vi "RenameVI.vi"(0 "ObjectIn":refnum<class "ClassWriterNative.lvclass">, 1 "VIItemRefIn":refnum<vi>, 2 "RenameOption":T1, 5 "error in (no error)":errorcluster) -> (14 "ObjectOut":refnum<class "ClassWriterNative.lvclass">, 19 "error out":errorcluster)   [LabVIEW 2020, in "ClassWriterNative.lvclass"]
uses:
  ClassWriterNative.lvclass
  Provider_BaseClassInterface/ClassWriter_class/RenameViOption.ctl
  <vilib>/picture/picture.llb/imagedata.ctl
  Provider_BaseClassInterface/ClassWriter_class/ClassWriter.lvclass
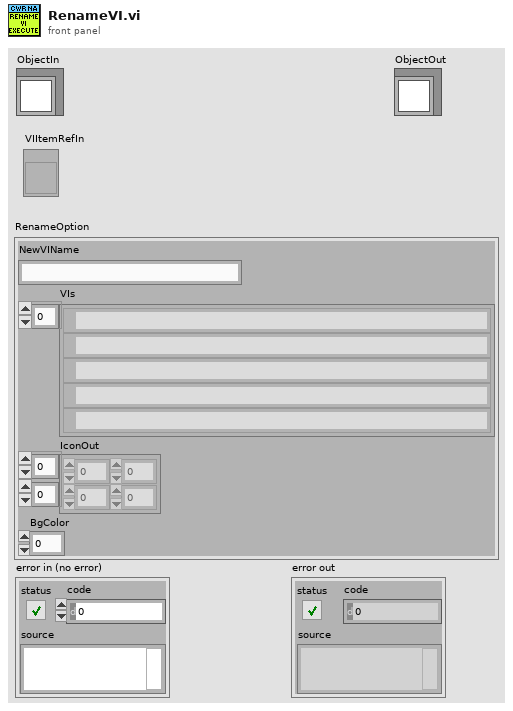
[diagram p1: front panel]
types:
  T1 = typedef "ClassWriter.lvclass/RenameViOption.ctl" = cluster{"NewVIName":string, "VIs":path[], "IconOut":u8[][], "BgColor":u8}
  T2 = cluster{"Counter":i32, "Text":string, "Cancelled":bool, "App Ref":refnum<vi>}
  T3 = typedef "imagedata.ctl" = cluster{"image type":i32, "image depth":i32, "image":u8[], "mask":u8[], "colors":u32[], "Rectangle":cluster{"left":i16, "top":i16, "right":i16, "bottom":i16}}
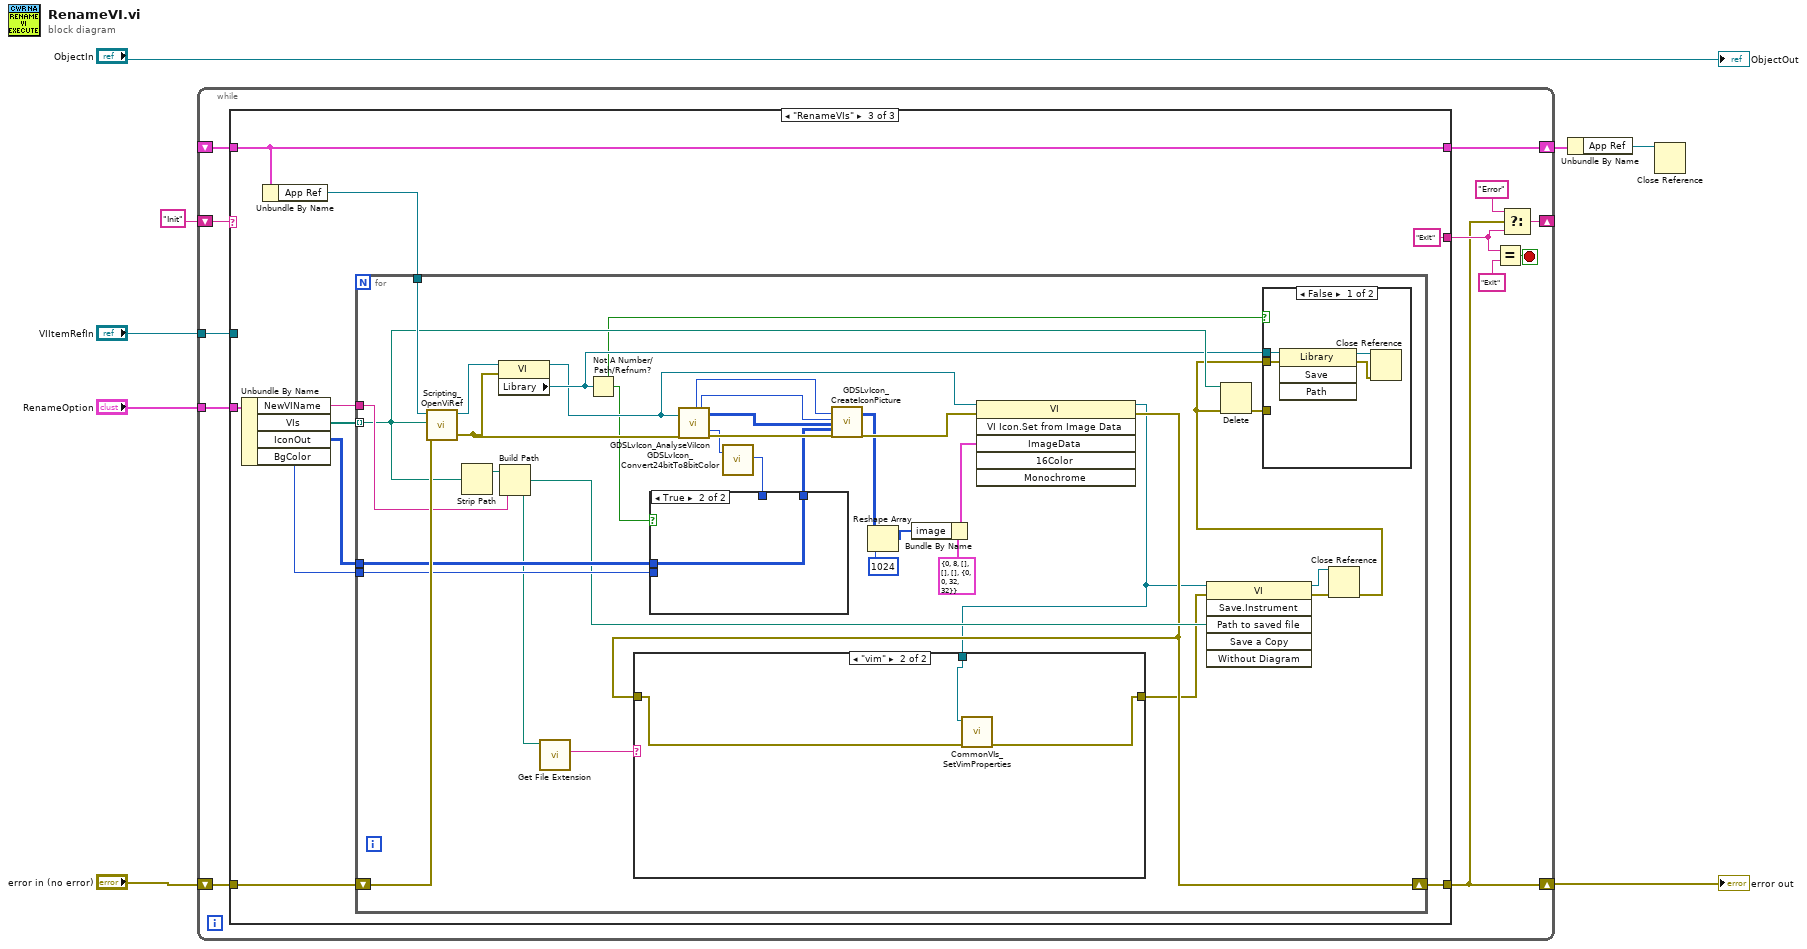
[diagram p0: block diagram]
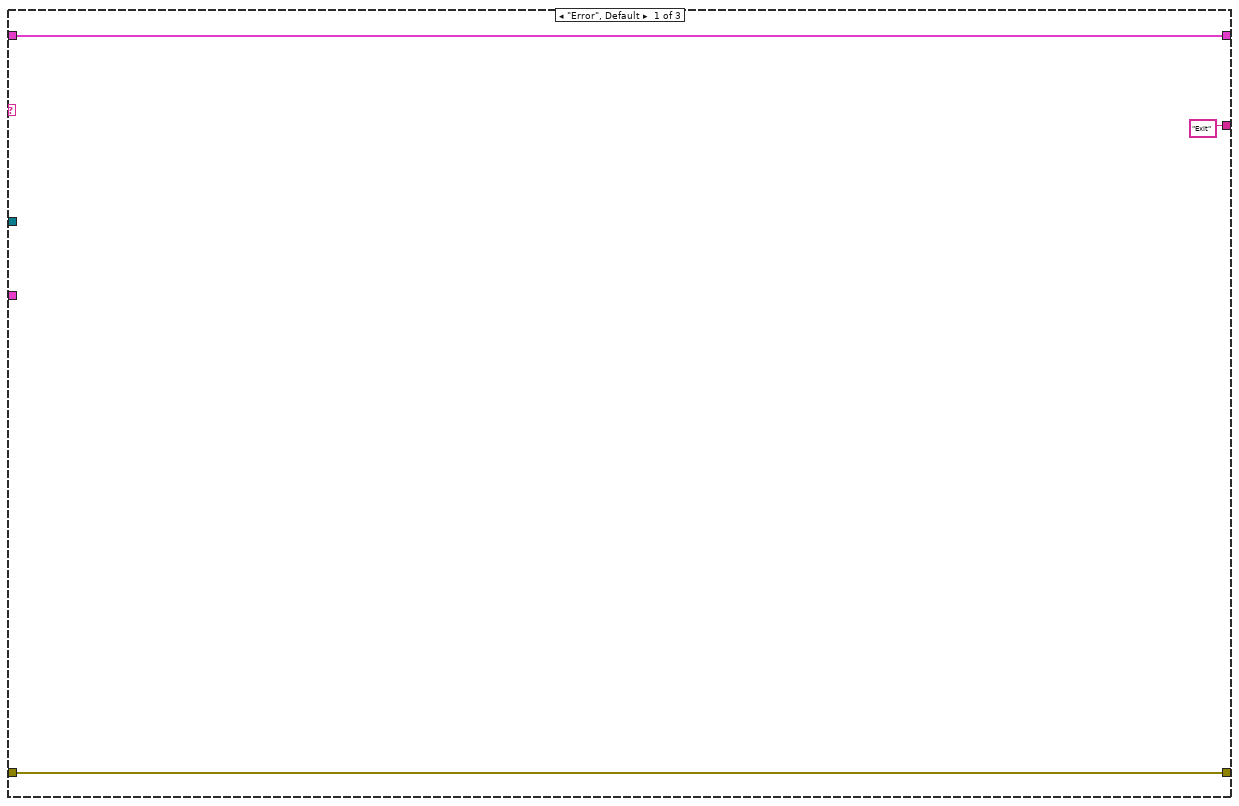
[diagram p2: hidden frame]
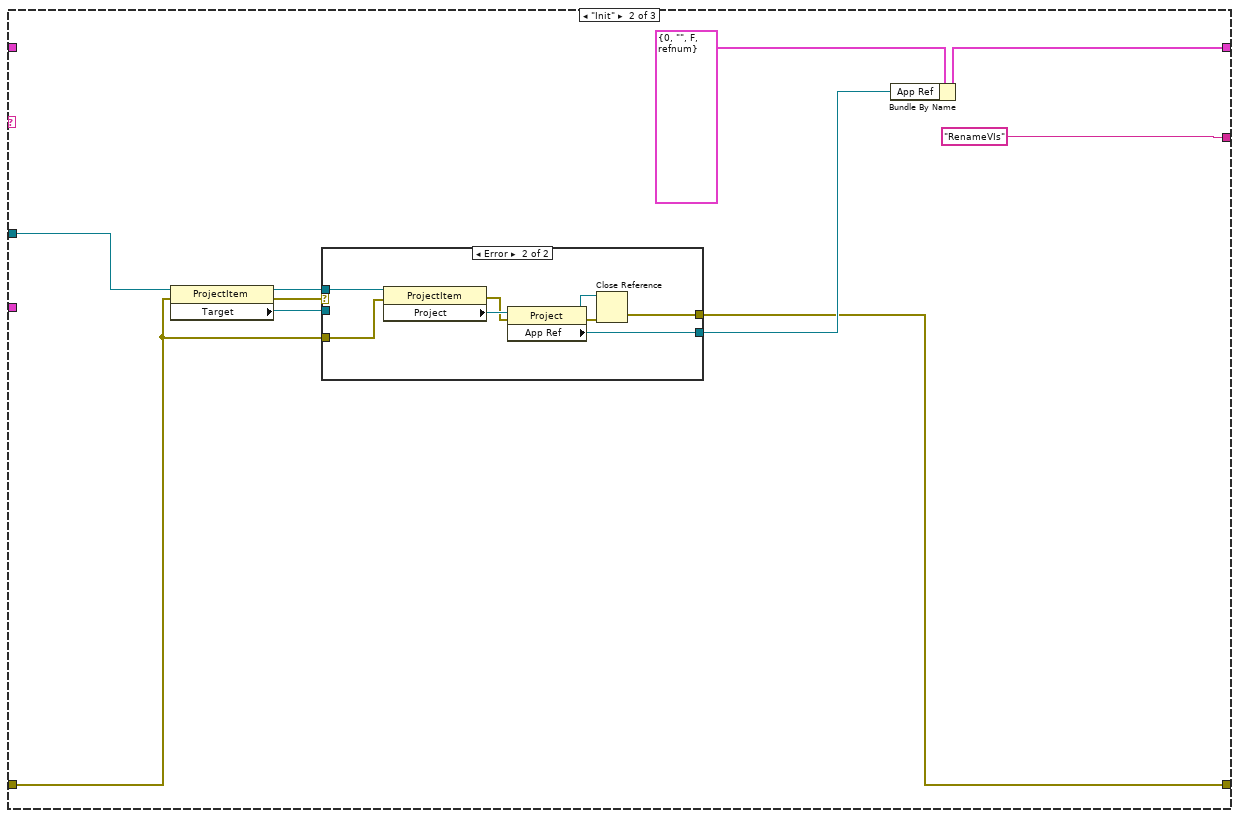
[diagram p3: hidden frame]
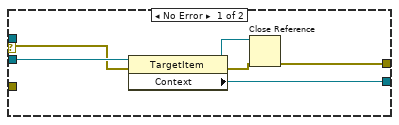
[diagram p4: hidden frame]
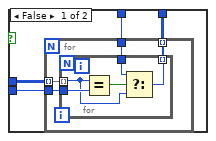
[diagram p6: hidden frame]
diagram:
  n1 = while {
    shift-right: [w13] -> w6
    shift-left: "error in (no error)" -> [w20]
    shift-right: [w18] -> _
    shift-left: "Init" -> [w19]
    shift-right: [w12] -> w8
    shift-left: _ -> [w11]
    tunnel: "RenameOption" -> [w10]
    tunnel: "VIItemRefIn" -> [w9]
    stop <- w17 stop-if-true
    n2 = case shown="\"RenameVIs\"" w19 {
      tunnel: w20 -> [w23 w25 w53]
      tunnel: [w23 w24 w52] -> w13
      tunnel: ["Exit" "RenameVIs" "Exit"] -> w14
      tunnel: [w21 w31 w56] -> w12
      tunnel: w11 -> [w21 _ w56]
      tunnel: w10 -> [_ _ w55]
      tunnel: w9 -> [_ w27 _]
      frame "Error", Default {
      }
      frame "Init" {
        n3 = property class="ProjectItem"(reference=w27, error in=w25) -> (reference out=w28:refnum<vi>, error out=w30:errorcluster, "Target"=w29:refnum<vi>)
        n4 = case shown="Error" w30 {
          selector: w30 -> [w35 _]
          tunnel: w29 -> [w39 _]
          tunnel: [w38 w41] -> w26
          tunnel: [w34 w42] -> w24
          tunnel: w28 -> [_ w47]
          tunnel: w25 -> [_ w46]
          frame No Error {
            n5 = property class="TargetItem"(reference=w39, error in=w35) -> (reference out=w36:refnum<vi>, error out=w37:errorcluster, "Context"=w38:refnum<vi>)
            n6 = Close Reference(reference=w36, error in (no error)=w37) -> (error out=w34:errorcluster)
          }
          frame Error {
            n7 = property class="ProjectItem"(reference=w47, error in=w46) -> (error out=w40:errorcluster, "Project"=w45:refnum<vi>)  [unwired: 1 out]
            n8 = property class="Project"(reference=w45, error in=w40) -> (reference out=w43:refnum<vi>, error out=w44:errorcluster, "App Ref"=w41:refnum<vi>)
            n9 = Close Reference(reference=w43, error in (no error)=w44) -> (error out=w42:errorcluster)
          }
        }
        n10 = Bundle By Name(cluster=T2 {"Counter"=0, "Text"="", "Cancelled"=FALSE, "App Ref"=refnum}, "App Ref"=w26) -> (w31:T2)
      }
      frame "RenameVIs" {
        n11 = Unbundle By Name(w55) -> ("NewVIName"=w51:string, "VIs"=w54:path[], "IconOut"=w50:u8[][], "BgColor"=w49:u8)
        n12 = Unbundle By Name(w56) -> ("App Ref"=w48:refnum<vi>)
        n13 = for {
          tunnel: w54 -> [w72] mode=indexing
          shift-right: [w60] -> w52
          shift-left: w53 -> [w91]
          tunnel: w51 -> [w89]
          tunnel: w50 -> [w80]
          tunnel: w49 -> [w79]
          tunnel: w48 -> [w75]
          n14 = call "Scripting_OpenViRef.vi"("error in"=w91, "ViPath/ViName/Viref"=w72, "AppRef"=w75) -> ("error out"=w65:errorcluster, "vi reference"=w71:refnum<vi>)  [unwired: 6 in, 1 out]
          n15 = Strip Path(path=w72) -> (stripped path=w90:path)  [unwired: 1 out]
          n16 = property class="VI"(reference=w71, error in=w65) -> (reference out=w64:refnum<vi>, "Library"=w69:refnum<vi>)  [unwired: 1 out]
          n17 = Build Path(base path=w90, name or relative path=w89) -> (appended path=w62:path)
          n18 = call <vilib>:"Get File Extension.vi"("file"=w62) -> ("lowercase file extension"=w61:string)  [unwired: 6 in, 4 out]
          n19 = Not A Number/Path/Refnum?(number/path/refnum=w69) -> (NaN/Path/Refnum?=w63:bool)
          n20 = call "GDSLvIcon_AnalyseViIcon.vi"("ViRef/LvCLassRef/LvLibRef/ViPath/2D_Image"=w64, "error in (no error)"=w65) -> ("FrameColor"=w74:u32, "FrameThickness(1)"=w73:u32, "HeaderIcon"=w81:u8[][], "BodyBkColor"=w77:u32, "error out"=w88:errorcluster)  [unwired: 5 in, 8 out]
          n21 = call "GDSLvIcon_Convert24bitTo8bitColor.vi"("Color 24bit In"=w77) -> ("Color out(256)"=w76:u8)  [unwired: 15 in, 3 out]
          n22 = case shown="True" w63 {
            tunnel: w80 -> [w99 w109]
            tunnel: w79 -> [w98 _]
            tunnel: [w97 w109] -> w78
            tunnel: w76 -> [w96 _]
            frame False {
              n23 = for {
                tunnel: w99 -> [w103] mode=indexing
                tunnel: w96 -> [w102]
                tunnel: w98 -> [w101]
                tunnel: [w100] -> w97 mode=indexing
                n24 = for {
                  tunnel: w103 -> [w104] mode=indexing
                  tunnel: w102 -> [w107]
                  tunnel: w101 -> [w105]
                  tunnel: [w106] -> w100 mode=indexing
                  n25 = Equal?(x=w104, y=w105) -> (x = y?=w108:bool)
                  n26 = Select(t=w107, s=w108, f=w104) -> (s? t:f=w106:u8)
                }
              }
            }
            frame True {
            }
          }
          n27 = call "GDSLvIcon_CreateIconPicture.vi"("FrameColor"=w74, "FrameThickness(1)"=w73, "HeaderIconIn"=w81, "BodyIconIn"=w78, "error in (no error)"=w88) -> ("WholeIconOut"=w82:u8[][], "error out"=w83:errorcluster)  [unwired: 9 in, 4 out]
          n28 = Reshape Array(w82, 1024 ("dimension size")) -> (w84:u8[])
          n29 = Bundle By Name(cluster=T3 {"image type"=0, "image depth"=8, "image"=[], "mask"=[], "colors"=[], "Rectangle"={"left"=0, "top"=0, "right"=32, "bottom"=32}} ("image data"), "image"=w84) -> (w85:T3)
          n30 = invoke class="VI" method="VI Icon.Set from Image Data"(reference=w64, error in=w83, "ImageData"=w85) -> (reference out=w58:refnum<vi>, error out=w60:errorcluster)  [unwired: 3 in, 4 out]
          n31 = case shown="\"vim\"" w61 {
            tunnel: w60 -> [w92 w95]
            tunnel: [w92 w93] -> w59
            tunnel: w58 -> [_ w94]
            frame Default {
            }
            frame "vim" {
              n32 = call "CommonVIs_SetVimProperties.vi"("error in (no error)"=w95, "VIRefIn"=w94) -> ("error out"=w93:errorcluster)  [unwired: 8 in, 1 out]
            }
          }
          n33 = invoke class="VI" method="Save.Instrument"(reference=w58, error in=w59, "Path to saved file"=w62) -> (reference out=w67:refnum<vi>, error out=w68:errorcluster)  [unwired: 3 in, 4 out]
          n34 = Close Reference(reference=w67, error in (no error)=w68) -> (error out=w66:errorcluster)
          n35 = Delete(path (use dialog)=w72, error in=w66) -> (error out=w70:errorcluster)  [unwired: 3 in, 2 out]
          n36 = case shown="False" w63 {
            tunnel: w70 -> [_ _]
            tunnel: w69 -> [w113 _]
            tunnel: w66 -> [w112 _]
            frame False {
              n37 = invoke class="Library" method="Save"(reference=w113, error in=w112) -> (reference out=w111:refnum<vi>, error out=w110:errorcluster)  [unwired: 2 in, 2 out]
              n38 = Close Reference(reference=w111, error in (no error)=w110) -> ()  [unwired: 1 out]
            }
            frame True {
            }
          }
        }
      }
    }
    n39 = Equal?(x=w14, y="Exit") -> (x = y?=w17:bool)
    n40 = Select(t="Error", s=w13, f=w14) -> (s? t:f=w18:string)
  }
  "error out" <- w6
  n41 = Unbundle By Name(w8) -> ("App Ref"=w1:refnum<vi>)
  n42 = Close Reference(reference=w1) -> ()  [unwired: 1 in, 1 out]
  "ObjectOut" <- "ObjectIn"
